vi "Test_C_W12_W13_W14.vi"() -> ()   [LabVIEW 2021]
uses:
  CANsub_C.lvlib
  C_Decode_Result.ctl
panel:
  out "length":i32
  out "echo frame":u8[](array[numeric]) format="%.0x"
  out "size data":i32
  out "id":u32[](array[numeric]) format="%.0x"
  out "data len":u8[](array[numeric])
  out "dlc":u8[](array[numeric])
  out "size hdlc":i32
  out "size ping":i32
  out "data":u8[](array[numeric])
  out "size ws":i32
  out "result":T1
  # "Expected values when run."
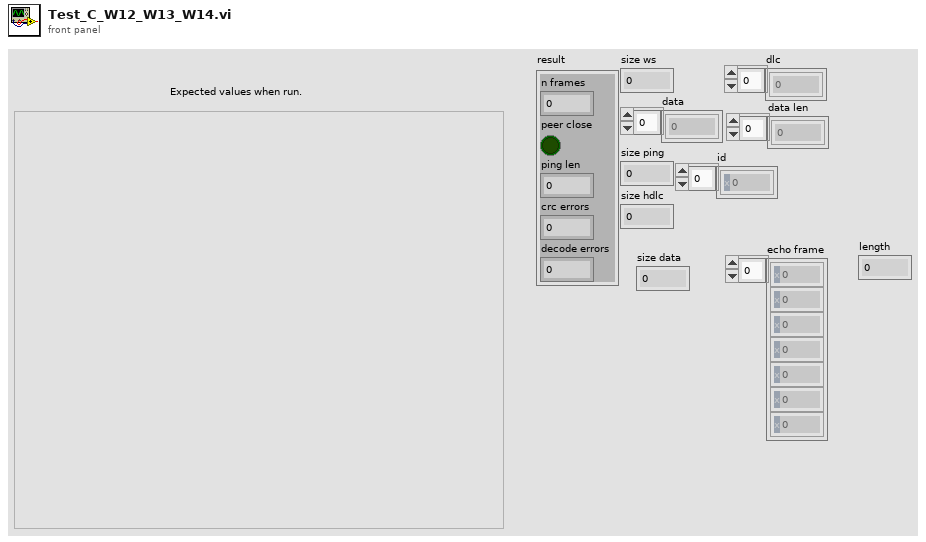
[diagram p1: front panel]
types:
  T1 = typedef "CANsub_C.lvlib/C_Decode_Result.ctl" = cluster{"n frames":i32, "peer close":bool, "ping len":i32, "crc errors":u32, "decode errors":i32}
  T2 = typedef "CANsub_C.lvlib/C_RX_Buffers.ctl" = cluster{"t_dev":dbl[], "ws":u8[], "id":u32[], "flags":u16[], "hdlc":u8[], "dlc":u8[], "data len":u8[], "data":u8[], "ping":u8[]}
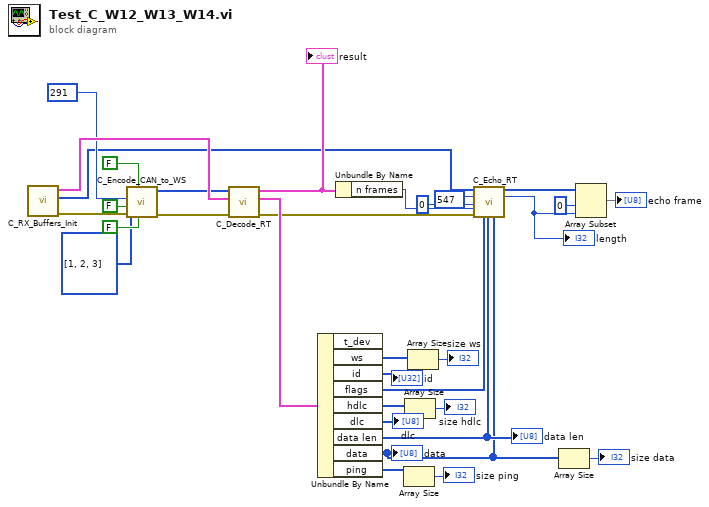
[diagram p0: block diagram]
diagram:
  n1 = call "C_RX_Buffers_Init.vi"() -> ("error out"=w31:errorcluster, "tx"=w1:u8[], "buffers"=w29:T2)  [unwired: 8 in, 1 out]
  n2 = call "C_Encode_CAN_to_WS.vi"("brs"=FALSE, "ide"=FALSE, "error in (no error)"=w31, "fdf"=FALSE, "id"=u32 291, "data"=u8[] [1, 2, 3]) -> ("error out"=w30:errorcluster, "ws frame"=w9:u8[])  [unwired: 4 in]
  n3 = call "C_Decode_RT.vi"("error in (no error)"=w30, "buffers in"=w29, "bytes in"=w9) -> ("error out"=w14:errorcluster, "buffers out"=w32:T2, "result"=w11:T1)  [unwired: 6 in]
  "result" <- w11
  n4 = Unbundle By Name(w32) -> ("ws"=w23:u8[], "id"=→"id":u32[], "flags"=w8:u16[], "hdlc"=w19:u8[], "dlc"=→"dlc":u8[], "data len"=w7:u8[], "data"=w6:u8[], "ping"=w21:u8[])  [unwired: 1 out]
  "data" <- w6
  "data len" <- w7
  n5 = Unbundle By Name(w11) -> ("n frames"=w10:i32)
  n6 = Array Size(array=w21) -> (size(s)=→"size ping":i32)
  n7 = Array Size(array=w19) -> (size(s)=→"size hdlc":i32)
  n8 = Array Size(array=w23) -> (size(s)=→"size ws":i32)
  n9 = call "C_Echo_RT.vi"("tx in"=w1, "flags"=w8, "data len"=w7, "data"=w6, "new id"=u32 547, "index"=0, "n frames"=w10, "error in (no error)"=w14) -> ("tx out"=w5:u8[], "length"=w4:i32)  [unwired: 5 in, 1 out]
  "length" <- w4
  n10 = Array Size(array=w6) -> (size(s)=→"size data":i32)
  n11 = Array Subset(array=w5, index=0, length=w4) -> (→"echo frame":u8[])
